vi "SetValueByItemIndex.vi"(0 "VI Reference In":refnum<vi>, 2 "delimiter (>>)":string=">>", 5 "Control Path":string, 7 "Item Index":i32, 11 "Error In":errorcluster) -> (4 "VI Reference Out":refnum<vi>, 15 "Error Out":errorcluster)   [LabVIEW 2016, in "Drona.lvlib" / "ControlValue.lvlib" / "StimulusListbox.lvlib"]
doc: "Sets value(signaling) for the listbox control whose index is specified. \n\nThe input control name is given as a string , incase of path, use delimiters inbetween the path."
uses:
  StimulusListbox.lvlib
  <vilib>/Utility/error.llb/Error Cluster From Error Code.vi
  <vilib>/ErrorRing/Error Ring.xnode
  Drona.lvlib
  Get/GetControlRef/GetControlRef.lvlib
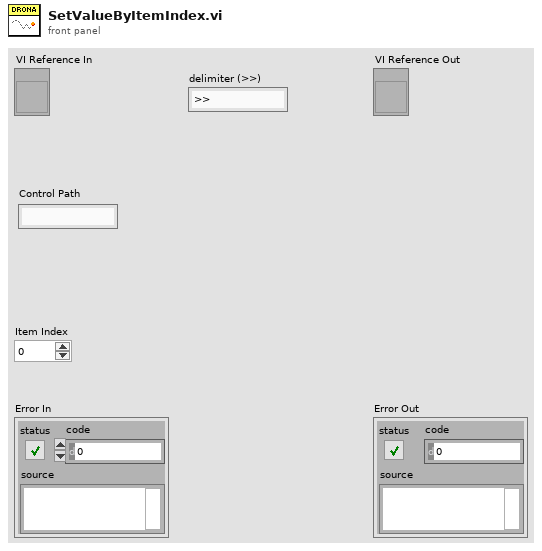
[diagram p1: front panel]
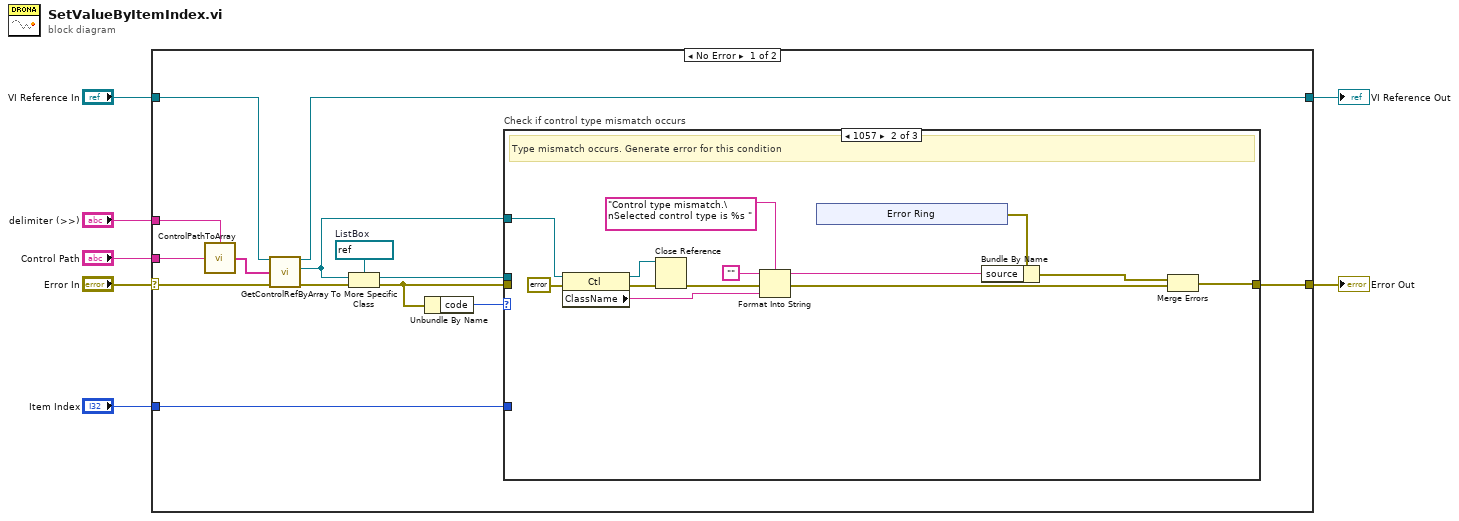
[diagram p0: block diagram]
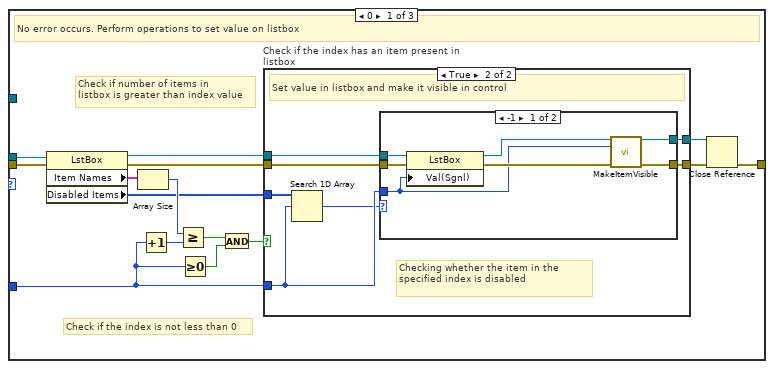
[diagram p2: hidden frame]
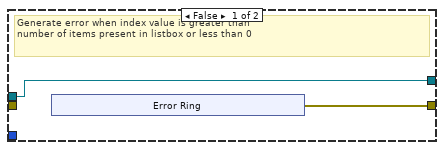
[diagram p3: hidden frame]
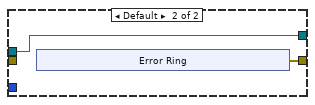
[diagram p4: hidden frame]
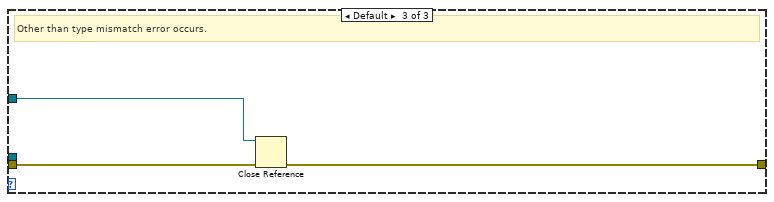
[diagram p5: hidden frame]
diagram:
  n1 = case shown="No Error" "Error In" {
    selector: "Error In" -> [w10 w87]
    tunnel: [w18 w87] -> w6
    tunnel: "VI Reference In" -> [w14 w86]
    tunnel: "Control Path" -> [w20 _]
    tunnel: "Item Index" -> [w16 _]
    tunnel: [w13 w86] -> w2
    tunnel: "delimiter (>>)" -> [w19 _]
    frame No Error {
      w21 = refnum<vi> refnum  # ListBox
      n2 = call "ControlPathToArray.vi"("Control Name"=w20, "delimiter (>>)"=w19) -> ("Control Path"=w15:string[])
      n3 = call "GetControlRefByArray.vi"("VI Reference In"=w14, "Control Path"=w15, "error In"=w10) -> ("VI Reference Out"=w13:refnum<vi>, "Ctl Refnum"=w11:refnum<vi>, "error out"=w12:errorcluster)  [unwired: 10 in]
      n4 = To More Specific Class(target class=w21, reference=w11, error in=w12) -> (specific class reference=w17:refnum<vi>, error out=w9:errorcluster)
      n5 = Unbundle By Name(w9) -> ("code"=w8:i32)
      n6 = case "Check if control type mismatch occurs" shown="1057" w8 {
        tunnel: [w36 w67 w84] -> w18
        tunnel: w17 -> [w28 _ _]
        tunnel: w16 -> [w26 _ _]
        tunnel: w11 -> [_ w77 w83]
        tunnel: w9 -> [w35 _ w85]
        frame 0 {
          # "Check if the index is not less than 0"
          # "Check if number of items in \nlistbox is greater than index value"
          # "No error occurs. Perform operations to set value on listbox"
          n7 = property class="LstBox"(reference=w28, error in=w35) -> (reference out=w27:refnum<vi>, error out=w32:errorcluster, "Item Names"=w31:string[], "Disabled Items"=w22:i32[])
          n8 = Array Size(array=w31) -> (size(s)=w30:i32)
          n9 = Increment(x=w26) -> (x+1=w29:i32)
          n10 = Greater Or Equal?(x=w30, y=w29) -> (x >= y?=w25:bool)
          n11 = Greater Or Equal To 0?(x=w26) -> (x >= 0?=w23:bool)
          n12 = And(x=w25, y=w23) -> (x .and. y?=w24:bool)
          n13 = case "Check if the index has an item present in listbox" shown="True" w24 {
            tunnel: [w37 w50] -> w34
            tunnel: [w38 w49] -> w33
            tunnel: w32 -> [_ w48]
            tunnel: w27 -> [w38 w47]
            tunnel: w26 -> [_ w45]
            tunnel: w22 -> [_ w46]
            frame False {
              # "Generate error when index value is greater than \nnumber of items present in listbox or less than 0"
              n14 = xnode "Error Ring"() -> ("error out"=w37:errorcluster)
            }
            frame True {
              # "Checking whether the item in the specified index is disabled"
              # "Set value in listbox and make it visible in control"
              n15 = Search 1D Array(1D array=w46, element=w45) -> (index of element=w44:i32)  [unwired: 1 in]
              n16 = case shown="-1" w44 {
                tunnel: [w57 w58] -> w50
                tunnel: [w56 w59] -> w49
                tunnel: w48 -> [w55 _]
                tunnel: w47 -> [w53 w59]
                tunnel: w45 -> [w52 _]
                frame -1 {
                  n17 = property class="LstBox"(reference=w53, error in=w55, "Val(Sgnl)"=w52) -> (reference out=w51:refnum<vi>, error out=w54:errorcluster)
                  n18 = call "MakeItemVisible.vi"("ListBox Ref In"=w51, "Item Index"=w52, "Error In"=w54) -> ("ListBox Ref Out"=w56:refnum<vi>, "Error Out"=w57:errorcluster)  [unwired: 11 in]
                }
                frame Default {
                  n19 = xnode "Error Ring"() -> ("error out"=w58:errorcluster)
                }
              }
            }
          }
          n20 = Close Reference(reference=w33, error in (no error)=w34) -> (error out=w36:errorcluster)
        }
        frame 1057 {
          # "Type mismatch occurs. Generate error for this condition"
          n21 = property class="Ctl"(reference=w77, error in=errorcluster {"status"=FALSE, "code"=0, "source"=""} ("error out")) -> (reference out=w65:refnum<vi>, error out=w76:errorcluster, "ClassName"=w73:string)
          n22 = Close Reference(reference=w65, error in (no error)=w76) -> (error out=w66:errorcluster)
          n23 = Format Into String(format string="Control type mismatch.\nSelected control type is %s ", initial string="", error in=w66, w73) -> (resulting string=w70:string, error out=w68:errorcluster)
          n24 = xnode "Error Ring"() -> ("error out"=w71:errorcluster)
          n25 = Bundle By Name(cluster=w71, "source"=w70) -> (w69:errorcluster)
          n26 = Merge Errors(w69, w68) -> (w67:errorcluster)
        }
        frame Default {
          # "Other than type mismatch error occurs."
          n27 = Close Reference(reference=w83, error in (no error)=w85) -> (error out=w84:errorcluster)
        }
      }
    }
    frame Error {
    }
  }
  "Error Out" <- w6
  "VI Reference Out" <- w2
